vi "VHist - Fit multi STR history to new timestamps.vi"(4 "merge data (T)":bool=TRUE, 6 "empty for absent (T)":bool=TRUE, 7 "new time stamps":dbl[](array[numeric]) format="%<%H:%M:%S%2u\n%d/%m/%Y>T", 8 "error in":errorcluster, 9 "time condition":cluster{"From":dbl, "To":dbl, "step, sec":dbl} {"step, sec" format="%.2f"; "To" format="%<%H:%M:%S%2u\n%d/%m/%Y>T"; "From" format="%<%H:%M:%S%2u\n%d/%m/%Y>T"}, 11 "history array":T1(array[cluster]) {"time stamps" format="%<%H:%M:%S%2u\n%d/%m/%Y>T"}) -> (0 "error out":errorcluster, 2 "multiple history data out":cluster{"history data":string[]}[](array[cluster]), 3 "time stamps out":dbl[](array[numeric]) format="%<%H:%M:%S%2u\n%d/%m/%Y>T")   [LabVIEW 2021]
doc: "The VI looks over several String histories and determines values of every history at the new common time stamps. New time stamps can be specified either in <b>new time stamps</b> array or <b>time conditions</b> cluster defining initial and final time, and time step. By default, VI replaces absent values with an empty string and merges values located between adjacent new time stamps. Either of these features can be suppressed.\n\nThe VI returns common time stamps in <b>time stamps out</b> array and history values in <b>multiple history data out</b> array. An element of <b>multiple history data out</b> is a cluster containing new history values for respective input history in <b>history array</b>.\n\n::: CalcExpress Toolkit :::\nCopyright (c) 2000-2026 Konstantin Shifershteyn. All rights reserved."
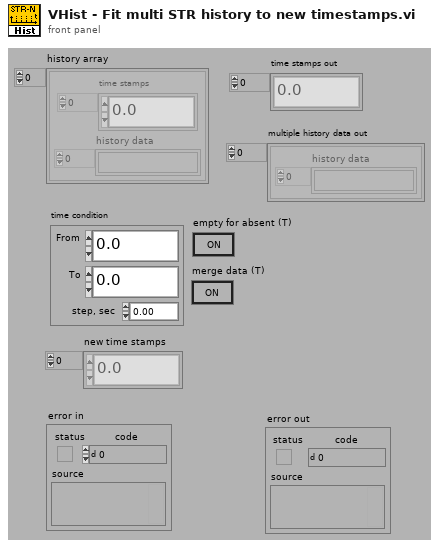
[diagram p1: front panel]
types:
  T1 = cluster{"time stamps":dbl[], "history data":string[]}[]
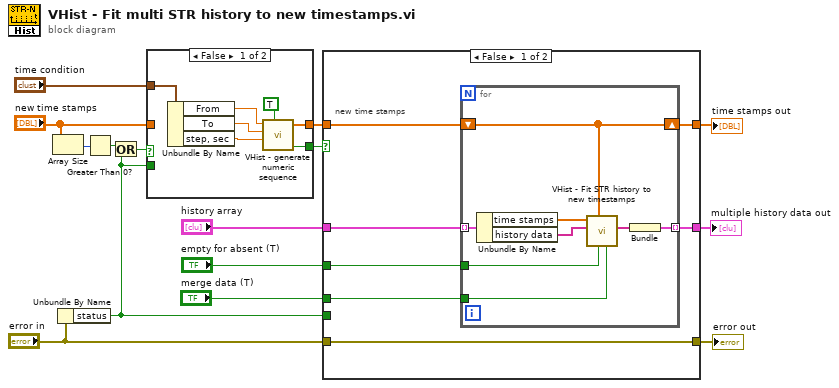
[diagram p0: block diagram]
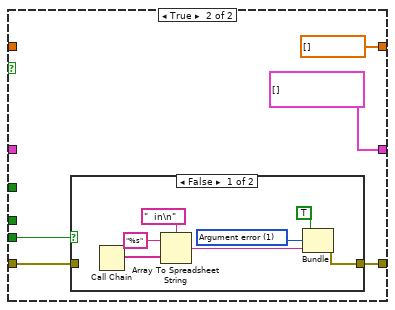
[diagram p3: hidden frame]
diagram:
  n1 = Array Size(array="new time stamps") -> (size(s)=w12:i32)
  n2 = Unbundle By Name("error in") -> ("status"=w7:bool)
  n3 = Greater Than 0?(x=w12) -> (x > 0?=w11:bool)
  n4 = Or(x=w11, y=w7) -> (x .or. y?=w10:bool)
  n5 = case shown="False" w10 {
    tunnel: [w21 w24] -> w5
    tunnel: "new time stamps" -> [_ w24]
    tunnel: "time condition" -> [w22 _]
    tunnel: [w16 w23] -> w6
    tunnel: w7 -> [_ w23]
    frame False {
      n6 = Unbundle By Name(w22) -> ("From"=w18:dbl, "To"=w19:dbl, "step, sec"=w20:dbl)
      n7 = call "VHist - generate numeric sequence.vi"("inclusive (T)"=TRUE, "step"=w20, "final value"=w19, "initial value"=w18) -> ("error"=w16:bool, "array out"=w21:dbl[])  [unwired: 4 in]
    }
    frame True {
    }
  }
  n8 = case shown="False" w6 {
    tunnel: [w31 cluster{string[]}[] []] -> w13
    tunnel: "error in" -> [w30 w43]
    tunnel: w7 -> [_ w44]
    tunnel: [w30 w42] -> w14
    tunnel: w5 -> [w29 _]
    tunnel: [w28 dbl[] []] -> w4
    tunnel: "merge data (T)" -> [w27 _]
    tunnel: "empty for absent (T)" -> [w26 _]
    tunnel: "history array" -> [w25 _]
    frame False {
      # "new time stamps"
      n9 = for {
        tunnel: w25 -> [w39] mode=indexing
        tunnel: [w38] -> w31 mode=indexing
        shift-right: [w32] -> w28
        shift-left: w29 -> [w32]
        tunnel: w26 -> [w35]
        tunnel: w27 -> [w34]
        n10 = Unbundle By Name(w39) -> ("time stamps"=w37:dbl[], "history data"=w36:string[])
        n11 = call "VHist - Fit STR history to new timestamps.vi"("merge data (T)"=w34, "empty for absent (T)"=w35, "new time stamps"=w32, "history data"=w36, "time stamps"=w37) -> ("history data out"=w33:string[])  [unwired: 4 in, 2 out]
        n12 = Bundle("history data out"=w33) -> (w38:cluster{"history data out":string[]})  [unwired: 1 in]
      }
    }
    frame True {
      n13 = case shown="False" w44 {
        tunnel: [w51 w52] -> w42
        tunnel: w43 -> [_ w52]
        frame False {
          w49 = 1 items=["No error", "Argument error", "Memory is full", "Out of zone", "End of file", "File already open", "Generic file I/O error", "File not found", "File permission error", "Disk is full", "Duplicate path", "Too many files open", "System feature not enabled", "Resource file not found", "Cannot add resource", "Resource not found", "Image not found", "Image memory error", "Pen does not exist", "Config type invalid", "Config token not found", "Config parse error", "Config memory error", "Bad external code format", "Bad external code offset", "External code not present", "Null window", "Destroy window error", "Null menu", "Print aborted", "Bad print record", "Print driver error", "Windows error during printing", "Memory error during printing", "Print dialog error", "Generic print error", "Invalid device refnum", "Device not found", "Device parameter error", "Device unit error", "Cannot open device", "Device call aborted", "Generic error", "Cancelled by user", "Object ID too low", "Object ID too high", "Object not in heap", "Unknown heap", "Unknown object (invalid DefProc)", "Unknown object (DefProc not in table)", "Message out of range", "Invalid (null) method", "Unknown message", "Manager call not supported", "Bad address", "Network operation in progress", "Network operation timed out", "Connection is busy", "Network attribute not supported", "Network error", "Address in use", "System out of memory", "Connection aborted", "Connection refused", "Not connected", "Already connected", "Connection closed", "Initialization error (interapplication manager)", "Bad occurrence", "Wait on unbound occurrence handler", "Occurrence queue overflow", "Datalog type conflict", "Unused", "Unrecognized type (interapplication manager)", "Memory corrupt", "Failed to make temporary DLL", "Old CIN version", "Drag socket not found", "Failed to load drop-object", "Failed to register OLE object", "Failed to release OLE object", "Format specifier type mismatch", "Unknown format specifier", "Too few format specifiers", "Too many format specifiers", "Scan failed", "Newer CIN version", "Error converting to variant", "Runtime menu error", "Password tampered", "Variant attribute not found", "Incompatible variant data type", "Event data is not available", "Event Store is not present", "Occurrence is not found", "Event Queue is not created", "Event info is not available", "Refnum passed is NULL", "Error retrieving Class GUID", "Error retrieving CoClass GUID", "Error retrieving TypeLib GUID.", "Bad built application magic bytes.", "Specific driver is different from the specific driver associated with the Logical Name.", "There is no session opened to the class driver.", "Max Error", "MAX - Error with config objects", "MAX - Error loading configuration", "MAX - Group not supported"]
          n14 = Call Chain() -> (call chain=w48:string[])
          n15 = Array To Spreadsheet String(delimiter (Tab)="  in\n", array=w48, 3:"%s" ("format string")) -> (spreadsheet string=w45:string)
          n16 = Bundle(TRUE, w49, "spreadsheet string"=w45) -> (w51:cluster{bool, i32, "spreadsheet string":string})  [unwired: 1 in]
        }
        frame True {
        }
      }
    }
  }
  "error out" <- w14
  "multiple history data out" <- w13
  "time stamps out" <- w4
